vi "Set Icon.vi"(8 "error in":errorcluster, 11 "ILabVIEWFile in":refnum<class "ILabVIEW File.lvclass">) -> (0 "error out":errorcluster, 3 "ILabVIEWFile out":refnum<class "ILabVIEW File.lvclass">)   [LabVIEW 2026, in "ILabVIEW File.lvclass"]
doc: "Set VI (or control) text icon using the name of the file from class private data."
uses:
  ILabVIEW File.lvclass
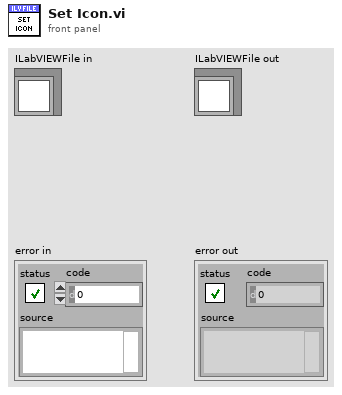
[diagram p1: front panel]
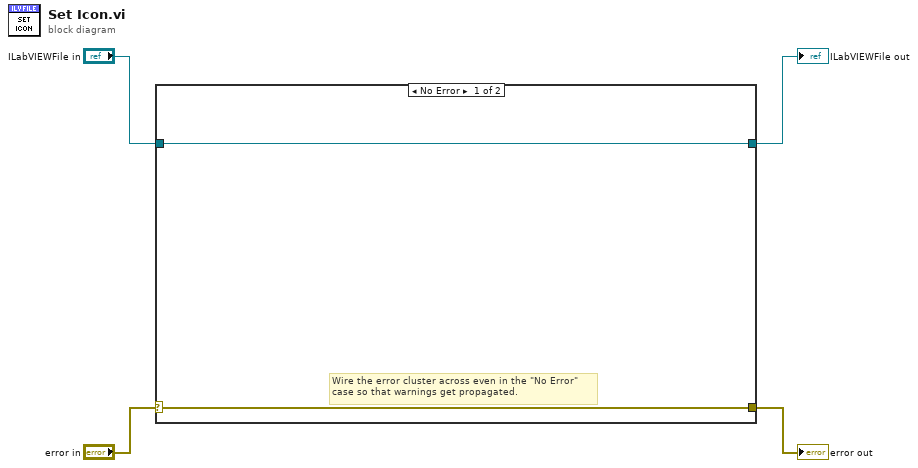
[diagram p0: block diagram]
diagram:
  n1 = case shown="No Error" "error in" {
    selector: "error in" -> [w6 w8]
    tunnel: [w6 w8] -> w3
    tunnel: [w5 w7] -> w1
    tunnel: "ILabVIEWFile in" -> [w5 w7]
    frame No Error {
      # "Wire the error cluster across even in the \"No Error\"\ncase so that warnings get propagated."
    }
    frame Error {
    }
  }
  "error out" <- w3
  "ILabVIEWFile out" <- w1
